vi "DiffDrvAccelLimit_Calculate.vi"(6 "RightVoltage":dbl, 8 "LeftVoltage":dbl, 9 "RightVelocity":dbl, 10 "LeftVelocity":dbl, 11 "inDiffDriveAccelLimit":T1) -> (0 "Error":bool, 2 "NewRightVoltage":dbl, 3 "NewLeftVoltage":dbl)   [LabVIEW 2019, in "Trajectory_Library.lvlib"]
doc: "Returns the next voltage pair subject to acceleraiton constraints.\n\nInputs:\n - DiffDriveAccelLimit -- Data cluster\n - leftVelocity -- The left wheel velocity in meters per second.\n - rightVelocity -- The right wheel velocity in meters per second.\n - leftVoltage -- The unconstrained left motor voltage.\n - rightVoltage -- The unconstrained right motor voltage.\n\nOutputs:\n - NewLeftVoltage -- The constraint drive left voltage output\n - NewRightVoltage -- The constraint drive right voltage output\n - Error -- If TRUE, an error occured."
uses:
  Trajectory_Library.lvlib
  <vilib>/Analysis/NI_AALBase.lvlib
  <vilib>/Analysis/baseanly.llb/Real A x B.vi
  <vilib>/Analysis/Matrix/NI_Matrix.lvlib
  <vilib>/Analysis/Matrix/Numeric/Add/Add - RM,RM.vi
  <vilib>/Analysis/NI_AALPro.lvlib
  <vilib>/Analysis/7linalg.llb/Solve Linear Equations (multiple right hand).vi
  <vilib>/Analysis/Matrix/Numeric/Subtract/Subtract - RM,RM.vi
  TypeDef/LINEAR_SYSTEM.ctl
  <vilib>/Analysis/Matrix/Datatypes/RealMatrix.ctl
  TypeDef/DIFF_DRIVE_ACCEL_LIMIT.ctl
panel:
  # "NOTE --- PERHAPS THE SYSTEM SHOULD NOT BE PART OF THE CLUSTER"
  # "<States,States>"
  # "<States,Inputs>"
  # "<Outputs,States>"
  # "<Outputs,Inputs>"
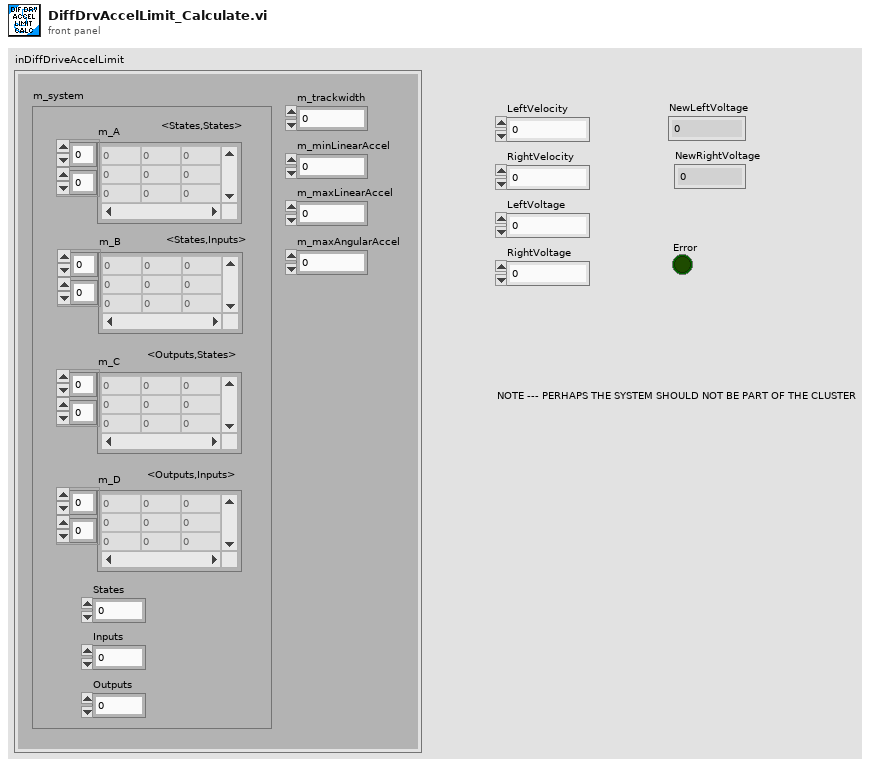
[diagram p1: front panel]
types:
  T1 = typedef "Trajectory_Library.lvlib/DIFF_DRIVE_ACCEL_LIMIT.ctl" = cluster{"m_system":T2, "m_trackwidth":dbl, "m_maxLinearAccel":dbl, "m_maxAngularAccel":dbl, "m_minLinearAccel":dbl}
  T2 = typedef "Trajectory_Library.lvlib/LINEAR_SYSTEM.ctl" = cluster{"m_A":T3, "m_B":T3, "m_C":T3, "m_D":T3, "States":i32, "Inputs":i32, "Outputs":i32}
  T3 = typedef "NI_Matrix.lvlib/RealMatrix.ctl" = dbl[][]
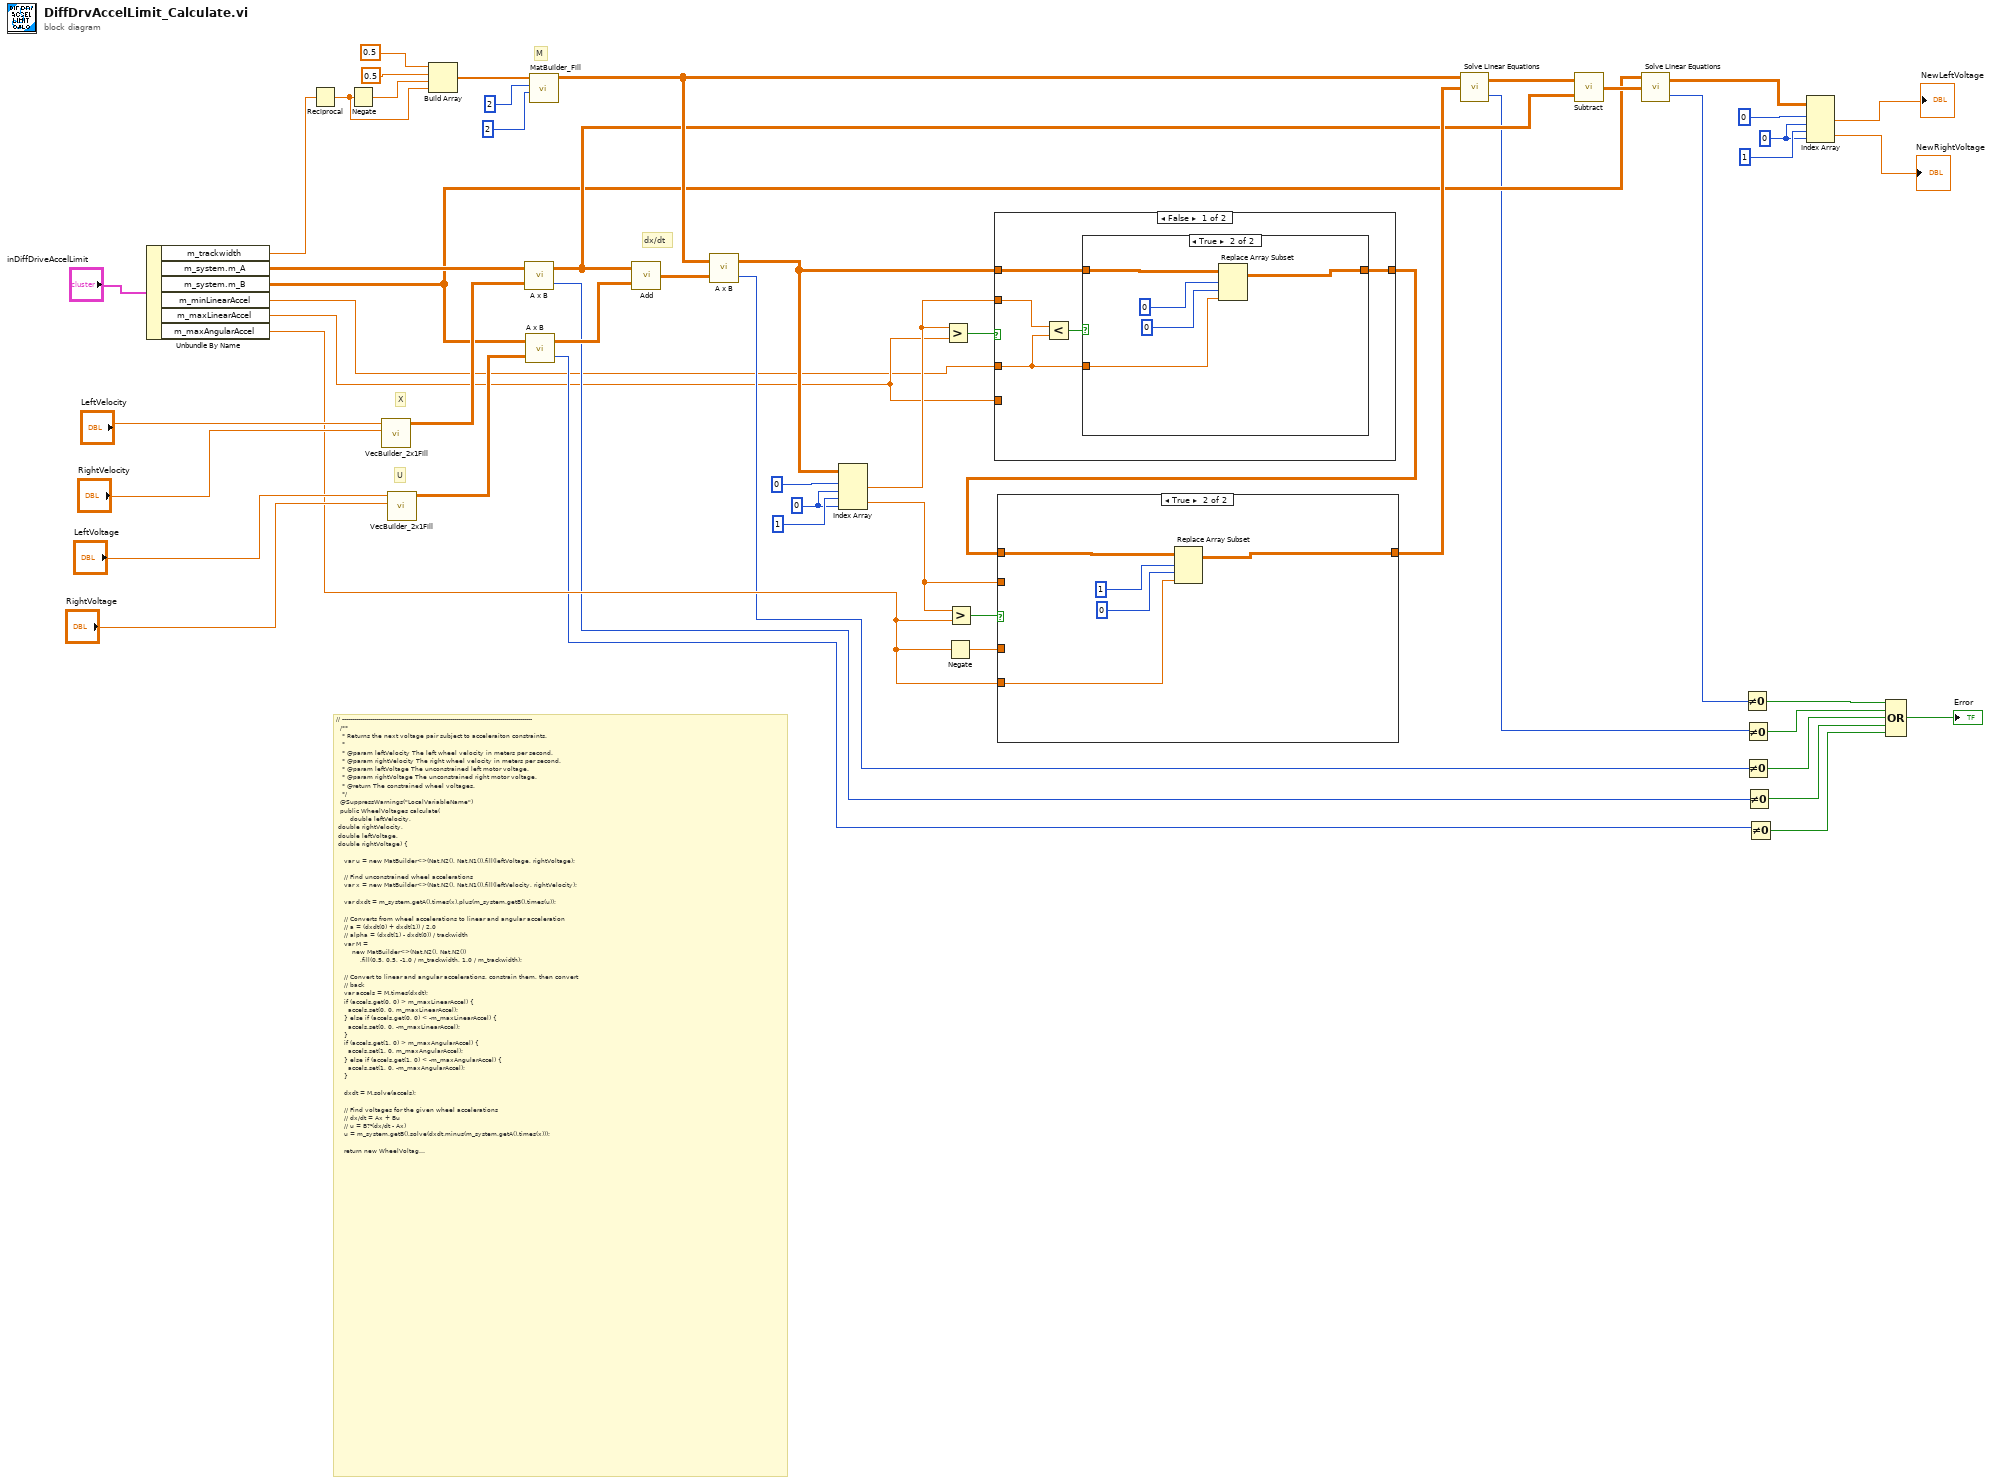
[diagram p0: block diagram]
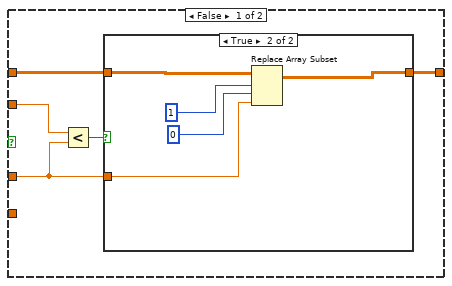
[diagram p2: hidden frame]
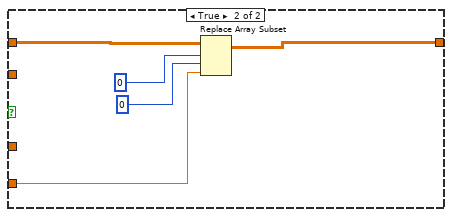
[diagram p5: hidden frame]
diagram:
  w23 = 0 ("index (col)")
  w35 = 0 ("index (col)")
  # "dx/dt"
  # "M"
  # "U"
  # "X"
  # "// -----------------------------------------------------------------------------------------------\n  /**\n   * Returns the next voltage pair subject to acceleraiton constraints.\n   *\n   * @param leftVelocity The left wheel velocity in meters per second.\n   * @param rightVelocity The right wheel velocity in meters per second.\n   * @param leftVoltage The unconstrained left motor voltage.\n   * @param rightVoltage The unconstrained right motor voltage.\n   * @return The constrained wheel voltages.\n   */\n  @SuppressWarnings(\"LocalVariableName\")\n  public WheelVoltages calculate(\n      \tdouble leftVelocity, \n\tdouble rightVelocity, \n\tdouble leftVoltage, \n\tdouble rightVoltage) {\n\n    var u = new MatBuilder<>(Nat.N2(), Nat.N1()).fill(leftVoltage, rightVoltage);\n\n    // Find unconstrained wheel accelerations\n    var x = new MatBuilder<>(Nat.N2(), Nat.N1()).fill(leftVelocity, rightVelocity);\n\n    var dxdt = m_system.getA().times(x).plus(m_system.getB().times(u));\n\n    // Converts from wheel accelerations to linear and angular acceleration\n    // a = (dxdt(0) + dxdt(1)) / 2.0\n    // alpha = (dxdt(1) - dxdt(0)) / trackwidth\n    var M =\n        new MatBuilder<>(Nat.N2(), Nat.N2())\n            .fill(0.5, 0.5, -1.0 / m_trackwidth, 1.0 / m_trackwidth);\n\n    // Convert to linear and angular accelerations, constrain them, then convert\n    // back\n    var accels = M.times(dxdt);\n    if (accels.get(0, 0) > m_maxLinearAccel) {\n      accels.set(0, 0, m_maxLinearAccel);\n    } else if (accels.get(0, 0) < -m_maxLinearAccel) {\n      accels.set(0, 0, -m_maxLinearAccel);\n    }\n    if (accels.get(1, 0) > m_maxAngularAccel) {\n      accels.set(1, 0, m_maxAngularAccel);\n    } else if (accels.get(1, 0) < -m_maxAngularAccel) {\n      accels.set(1, 0, -m_maxAngularAccel);\n    }\n\n    dxdt = M.solve(accels);\n\n    // Find voltages for the given wheel accelerations\n    // dx/dt = Ax + Bu\n    // u = B?¹(dx/dt - Ax)\n    u = m_system.getB().solve(dxdt.minus(m_system.getA().times(x)));\n\n    return new WheelVoltages(u.get(0, 0), u.get(1, 0));\n  }"
  n1 = Unbundle By Name("inDiffDriveAccelLimit") -> ("m_trackwidth"=w3:dbl, "m_system.m_A"=w49:T3, "m_system.m_B"=w18:T3, "m_minLinearAccel"=w1:dbl, "m_maxLinearAccel"=w2:dbl, "m_maxAngularAccel"=w19:dbl)
  n2 = Reciprocal(x=w3) -> (1/x=w39:dbl)
  n3 = Negate(x=w39) -> (-x=w40:dbl)
  n4 = call "VecBuilder_2x1Fill.vi"("R1"="RightVelocity", "R0"="LeftVelocity") -> ("output matrix"=w48:T3)  [unwired: 9 in]
  n5 = call "VecBuilder_2x1Fill.vi"("R1"="RightVoltage", "R0"="LeftVoltage") -> ("output matrix"=w47:T3)  [unwired: 9 in]
  n6 = Build Array(0.5 ("element"), 0.5 ("element"), w40, w39) -> (w45:dbl[])
  n7 = call-poly <vilib>:"A x B.vi"("B"=w48, "A"=w49) -> ("error"=w11:i32, "A x B"=w21:T3)
  n8 = call-poly <vilib>:"A x B.vi"("B"=w47, "A"=w18) -> ("error"=w10:i32, "A x B"=w46:T3)
  n9 = call "MatBuilder_Fill.vi"("Columns"=2, "Rows"=2, "Value List"=w45) -> ("output matrix"=w27:T3)  [unwired: 8 in]
  n10 = call-poly <vilib>:"Add.vi"("Real Matrix B"=w46, "Real Matrix A"=w21) -> ("A + B"=w38:T3)
  n11 = call-poly <vilib>:"A x B.vi"("B"=w38, "A"=w27) -> ("error"=w12:i32, "A x B"=w32:T3)
  n12 = Index Array(array=w32, index (row) #1=0 ("index (row)"), index (col) #1=w35, index (row) #2=1 ("index (row)"), index (col) #2=w35) -> (element #1=w33:dbl, element #2=w29:dbl)
  n13 = Greater?(x=w33, y=w2) -> (0:w34:bool)
  n14 = Negate(x=w19) -> (-x=w30:dbl)
  n15 = Greater?(x=w29, y=w19) -> (0:w31:bool)
  n16 = case shown="False" w34 {
    tunnel: w33 -> [w58 _]
    tunnel: w1 -> [w55 _]
    tunnel: w32 -> [w57 w70]
    tunnel: [w56 w66] -> w28
    tunnel: w2 -> [_ w67]
    frame False {
      n17 = Less?(x=w58, y=w55) -> (x < y?=w59:bool)
      n18 = case shown="True" w59 {
        tunnel: w57 -> [w60 w62]
        tunnel: [w60 w61] -> w56
        tunnel: w55 -> [_ w63]
        frame False {
        }
        frame True {
          n19 = Replace Array Subset(array=w62, new element=w63, index (row)=0 ("disabled index (row)"), index (col)=0 ("disabled index (col)")) -> (w61:T3)
        }
      }
    }
    frame True {
      n20 = Replace Array Subset(array=w70, new element=w67, index (row)=0 ("disabled index (row)"), index (col)=0 ("disabled index (col)")) -> (w66:T3)
    }
  }
  n21 = case shown="True" w31 {
    tunnel: w29 -> [w74 _]
    tunnel: w30 -> [w71 _]
    tunnel: w28 -> [w73 w86]
    tunnel: [w72 w82] -> w26
    tunnel: w19 -> [_ w83]
    frame False {
      n22 = Less?(x=w74, y=w71) -> (x < y?=w75:bool)
      n23 = case shown="True" w75 {
        tunnel: w73 -> [w76 w78]
        tunnel: [w76 w77] -> w72
        tunnel: w71 -> [_ w79]
        frame False {
        }
        frame True {
          n24 = Replace Array Subset(array=w78, new element=w79, index (row)=1 ("disabled index (row)"), index (col)=0 ("disabled index (col)")) -> (w77:T3)
        }
      }
    }
    frame True {
      n25 = Replace Array Subset(array=w86, new element=w83, index (row)=1 ("disabled index (row)"), index (col)=0 ("disabled index (col)")) -> (w82:T3)
    }
  }
  n26 = call-poly <vilib>:"Solve Linear Equations.vi"("Known Matrix"=w26, "Input Matrix"=w27) -> ("error"=w13:i32, "Solution Matrix"=w22:T3)  [unwired: 1 in]
  n27 = call-poly <vilib>:"Subtract.vi"("Real Matrix B"=w21, "Real Matrix A"=w22) -> ("A - B"=w20:T3)
  n28 = call-poly <vilib>:"Solve Linear Equations.vi"("Known Matrix"=w20, "Input Matrix"=w18) -> ("error"=w14:i32, "Solution Matrix"=w17:T3)  [unwired: 1 in]
  n29 = Not Equal To 0?(x=w14) -> (x != 0?=w9:bool)
  n30 = Not Equal To 0?(x=w13) -> (x != 0?=w8:bool)
  n31 = Not Equal To 0?(x=w12) -> (x != 0?=w7:bool)
  n32 = Not Equal To 0?(x=w11) -> (x != 0?=w6:bool)
  n33 = Not Equal To 0?(x=w10) -> (x != 0?=w5:bool)
  n34 = Index Array(array=w17, index (row) #1=0 ("index (row)"), index (col) #1=w23, index (row) #2=1 ("index (row)"), index (col) #2=w23) -> (element #1=→"NewLeftVoltage":dbl, element #2=→"NewRightVoltage":dbl)
  n35 = Compound Arithmetic op=OR(w9, w8, w7, w6, w5) -> (→"Error":bool)
